vi "bring_to_initial_position__d0a7d68fce.vi"(0 "Refnum in":refnum<k21>, 1 "Initial position in Voltage (V) in":dbl, 5 "Initial PID gains":T1, 7 "instrument handle in":refnum<k15>, 9 "Array in":string[](array[string]), 11 "error in (no error)":errorcluster, 12 "error in":errorcluster) -> (2 "instrument handle out":refnum<k15>, 3 "status":bool, 4 "Refnum out":refnum<k21>, 6 "error out 3":errorcluster, 8 "status 2":bool, 10 "Boolean":bool, 14 "Array out":string[](array[string]), 15 "error out":errorcluster)   [LabVIEW 2023]
uses:
  <vilib>/DAQmx/read.llb/DAQmx Read (Analog DBL 1Chan 1Samp).vi
  <vilib>/DAQmx/miscellaneous.llb/DAQmx Fill In Error Info.vi
  <vilib>/addons/control/pid/pid.llb/PID Advanced (DBL).vi
  <vilib>/addons/control/pid/NI_PID_pid.lvlib
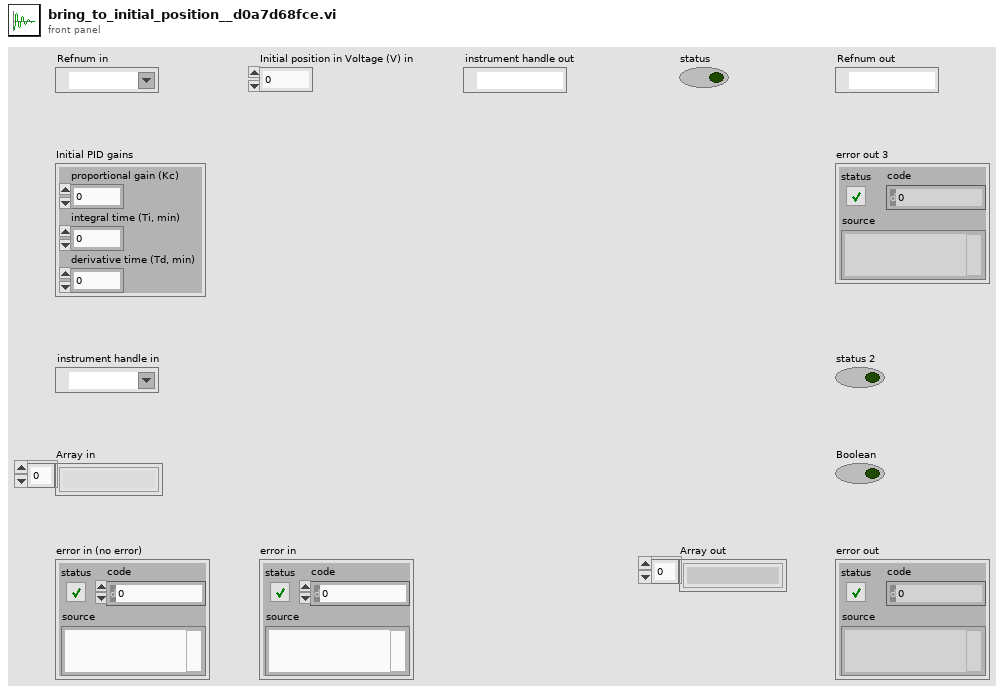
[diagram p1: front panel]
types:
  T1 = cluster{"proportional gain (Kc)":dbl, "integral time (Ti, min)":dbl, "derivative time (Td, min)":dbl}
  T2 = typedef "LVDateTimeRec.ctl" = cluster{"fractional second":dbl, "second":i32, "minute":i32, "hour":i32, "day of month":i32, "month":i32, "year":i32, "day of week":i32, "day of year":i32, "DST":i32}
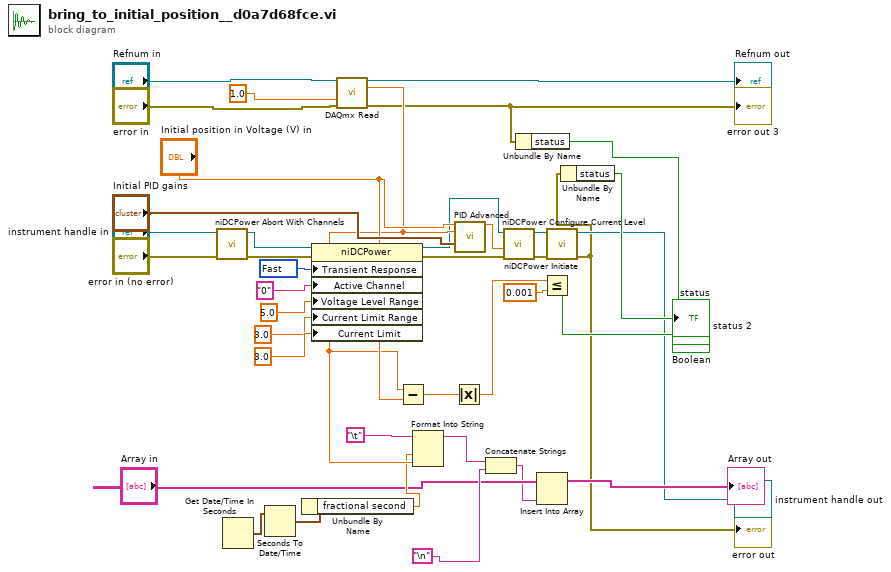
[diagram p0: block diagram]
diagram:
  w3 = 1039 items=["Slow"=1041, "Normal"=1038, "Fast"=1039, "Custom"=1042] ("Source:Transient Response")
  n1 = call <instrlib>:"niDCPower Abort With Channels.vi"("error in (no error)"="error in (no error)", "instrument handle"="instrument handle in") -> ("error out"=w8:errorcluster, "instrument handle out"=w7:refnum<k15>)  [unwired: 8 in]
  n2 = Get Date/Time In Seconds() -> (seconds since 1Jan1904=w30:timestamp)
  n3 = Seconds To Date/Time(time stamp (now)=w30) -> (date time rec=w29:T2)  [unwired: 1 in]
  n4 = Unbundle By Name(w29) -> ("fractional second"=w31:dbl)
  n5 = property class="niDCPower"(reference=w7, error in=w8, "Transient Response"=w3, "Active Channel"="0", "Voltage Level Range"=5.0 ("Source:DC Voltage:Voltage Level Range"), "Current Limit Range"=3.0 ("Source:DC Voltage:Current Limit Range"), "Current Limit"=3.0 ("Source:DC Voltage:Current Limit")) -> (reference out=w9:refnum<k15>, error out=w10:errorcluster)
  n6 = call-poly <vilib>:"DAQmx Read.vi"("task/channels in"="Refnum in", "timeout"=1.0, "error in"="error in") -> ("task out"=→"Refnum out":refnum<k21>, "data"=w32:dbl, "error out"=w20:errorcluster)  [unwired: 10 in]
  "error out 3" <- w20
  n7 = Subtract(x=w32, y="Initial position in Voltage (V) in") -> (x-y=w17:dbl)
  n8 = Format Into String(initial string="\t", w31, w32) -> (resulting string=w23:string)  [unwired: 2 in, 1 out]
  n9 = Absolute Value(x=w17) -> (abs(x)=w18:dbl)
  n10 = call-poly <vilib>:"PID Advanced.vi"("setpoint"="Initial position in Voltage (V) in", "process variable"=w32, "PID gains"="Initial PID gains") -> ("output"=w16:dbl)  [unwired: 11 in, 1 out]
  n11 = Concatenate Strings(w23, "\n") -> (w25:string)
  n12 = call <instrlib>:"niDCPower Configure Current Level.vi"("error in (no error)"=w10, "current level"=w16, "instrument handle"=w9) -> ("error out"=w12:errorcluster, "instrument handle out"=w11:refnum<k15>)  [unwired: 7 in]
  n13 = Unbundle By Name(w20) -> ("status"=→"status 2":bool)
  n14 = Insert Into Array(array="Array in", new element=w25) -> (→"Array out":string[])  [unwired: 1 in]
  n15 = Less Or Equal?(x=w18, y=0.001) -> (x <= y?=→"Boolean":bool)
  n16 = call <instrlib>:"niDCPower Initiate.vi"("error in (no error)"=w12, "instrument handle"=w11) -> ("error out"=w21:errorcluster, "instrument handle out"=→"instrument handle out":refnum<k15>)  [unwired: 2 in, 6 out]
  "error out" <- w21
  n17 = Unbundle By Name(w21) -> ("status"=→"status":bool)
